vi "CSE - Execute Script (Basic).vi"(4 "Breakpoints":i32[](array[numeric]), 6 "exec parameters":T3={"pause counter"=1000, "pause, ms"=0, "autoVar"=TRUE, "enCpx"=TRUE}, 7 "VC Handle":T6=-1, 8 "error in":errorcluster, 9 "Run mode":T2 items=["Execute", "Abort", "Run", "Step", "Step Over", "Step Out", "Run (LM)", "Step (LM)", "Step Over (LM)", "Step Out (LM)", "unsupported"], 10 "Stm Index":i32, 11 "CSE RefNum":T4) -> (0 "error out":errorcluster, 1 "Stop Reason":T1=1 items=["Exec Start", "Action completed", "pause to breath", "reserved 1", "reserved 2", "custom"], 2 "Stm Index out":i32, 3 "dup CSE RefNum":T4, 5 "return value":dbl)   [LabVIEW 2021]
doc: "This VI is the basic CSE script executor. You can use it to run a parsed script, or you can create your own script engine based on it. Refer to the VI help for more details.\n\nIf <b>Run mode</b> is 0 (Execute), the VI completely executes a script starting from the <b>Stm Index</b> position (statement index) in regular mode with debugging disabled. Otherwise, the VI stops if either the specified action is completed or a breakpoint is reached.\n\n<b>Stm Index</b> specifies the initial index of the statement in a parsed script to execute.\n\n<b>Stm Index out</b> indicator returns the index of the statement to be performed next. When a script completes, <b>Stm Index out</b> returns -1.\n\n<b>Stop Reason</b> indicates the reason for the VI stop. The VI can return either 1 (Action completed) or 2 (pause to breath). All other values are reserved for compatibility with the \"Call Reason\" control of a Callback VI.\n\n<b>NOTE</b>: This VI never finishes until it completely executes a statement; it cannot return in the middle of a statement processing. This is true even if a statement involves calls to FuncVI functions.\n\n::: CalcExpress Toolkit :::\nCopyright (c) 2000-2026 Konstantin Shifershteyn. All rights reserved."
uses:
  cetypes.llb/VarMan Variable Context Handle.ctl
  cetypes.llb/CalcExpress Instance RefNum.ctl
  CSE Instance RefNum.ctl
  CSE Type - Run Mode.ctl
  CSE Type - Callback Call Reason.ctl
  cersrc/celveng32.dll
panel:
  in  "CE RefNum Tmpl":T5
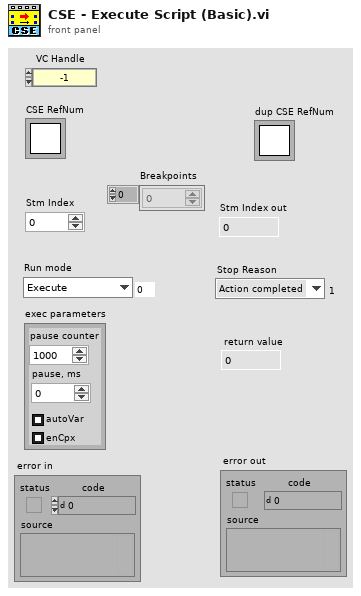
[diagram p1: front panel]
types:
  T1 = typedef "CSE Type - Callback Call Reason.ctl" = u32
  T2 = typedef "CSE Type - Run Mode.ctl" = u32
  T3 = cluster{"pause counter":i32, "pause, ms":i32, "autoVar":bool, "enCpx":bool}
  T4 = typedef "CSE Instance RefNum.ctl" = refnum<k1>
  T5 = typedef "CalcExpress Instance RefNum.ctl" = refnum<k1>
  T6 = typedef "VarMan Variable Context Handle.ctl" = i32
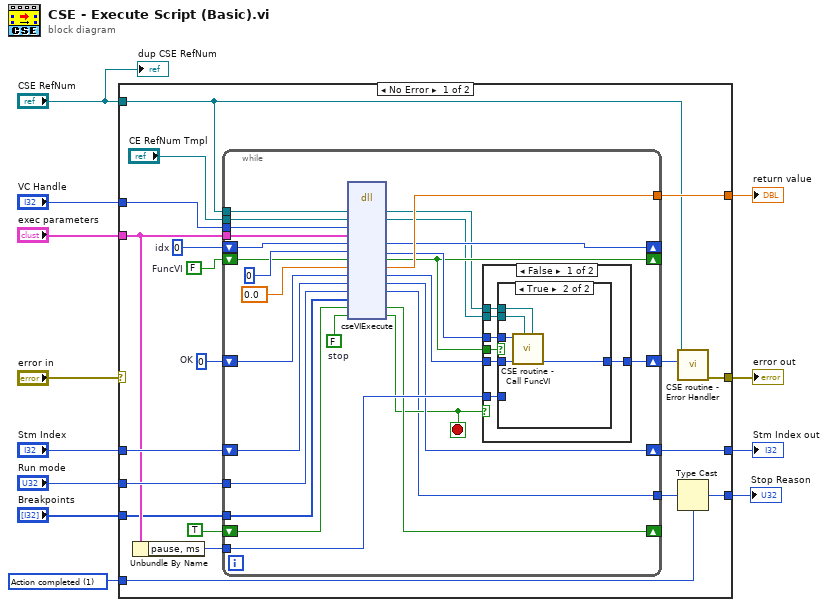
[diagram p0: block diagram]
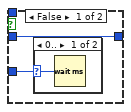
[diagram p2: hidden frame]
diagram:
  w1 = T1 1 items=["Exec Start", "Action completed", "pause to breath", "reserved 1", "reserved 2", "custom"] ("Stop Reason")
  n1 = case shown="No Error" "error in" {
    selector: "error in" -> [_ w77]
    tunnel: "VC Handle" -> [w30 _]
    tunnel: [w29 _] -> w11
    tunnel: [w28 w76] -> w10
    tunnel: "Stm Index" -> [w27 w76]
    tunnel: "CSE RefNum" -> [w20 _]
    tunnel: "Run mode" -> [w23 _]
    tunnel: "exec parameters" -> [w22 _]
    tunnel: [w19 w77] -> w5
    tunnel: "Breakpoints" -> [w16 _]
    tunnel: [w14 w75] -> w2
    tunnel: w1 -> [w13 w75]
    frame No Error {
      w24 = FALSE  # FuncVI
      w26 = 0  # OK
      w31 = 0  # idx
      n2 = Unbundle By Name(w22) -> ("pause, ms"=w25:i32)
      n3 = while {
        shift-left: w27 -> [w45]
        shift-right: [w43] -> w28
        tunnel: [w50] -> w29
        tunnel: w20 -> [w52]
        tunnel: w30 -> [w54]
        tunnel: "CE RefNum Tmpl" -> [w53]
        tunnel: w22 -> [w42]
        shift-left: w31 -> [w41]
        shift-right: [w40] -> _
        shift-left: w26 -> [w57]
        shift-right: [w58] -> w21
        tunnel: w25 -> [w48]
        shift-right: [w46] -> _
        shift-left: w24 -> [w47]
        tunnel: w23 -> [w44]
        shift-right: [w37] -> _
        shift-left: TRUE -> [w39]
        tunnel: w16 -> [w35]
        tunnel: [w34] -> w15
        stop <- w36 stop-if-true
        w38 = FALSE  # stop
        n4 = dll-call lib="C:/LV Projects/CalcExpress 40 LV2021/vi.lib/addons/CalcExpress/cersrc/celveng*.dll" fn="cseVIExecute" ("viCESPExecute")("iCESP"=w52, "iCE"=w53, "vch"=w54, "ExecPars"=w42, "expIdx"=w41, "expPNum"=0, "FuncVI"=w47, "retVal"=0.0 ("numeric value"), "ExecStat"=w57, "StmIdx"=w45, "Mode/Reason"=w44, "bpArray"=w35, "FirstTime"=w39, "stop"=w38) -> ("iCESP"=w32:T4, "iCE"=w33:T5, "expIdx"=w40:i32, "expPNum"=w49:i32, "FuncVI"=w46:bool, "retVal"=w50:dbl, "ExecStat"=w51:i32, "StmIdx"=w43:i32, "Mode/Reason"=w34:T2, "FirstTime"=w37:bool, "stop"=w36:bool)  [unwired: 7 in, 2 out]
        n5 = case shown="False" w36 {
          tunnel: [w65 w74] -> w58
          tunnel: w51 -> [w64 w74]
          tunnel: w49 -> [w63 _]
          tunnel: w46 -> [w62 _]
          tunnel: w48 -> [w61 _]
          tunnel: w33 -> [w60 _]
          tunnel: w32 -> [w59 _]
          frame False {
            n6 = case shown="True" w62 {
              tunnel: [w67 w71] -> w65
              tunnel: w64 -> [w67 w72]
              tunnel: w63 -> [_ w73]
              tunnel: w61 -> [w66 _]
              tunnel: w60 -> [_ w70]
              tunnel: w59 -> [_ w69]
              frame False {
                n7 = case shown="0.." w66 {
                  selector: w66 -> [w68 _]
                  frame 0.. {
                    n8 = Wait (ms)(milliseconds to wait=w68) -> ()  [unwired: 1 out]
                  }
                  frame ..-1 {
                  }
                }
              }
              frame True {
                n9 = call "CSE routine - Call FuncVI.vi"("CSE RefNum"=w69, "CE InstanceRef"=w70, "error code"=w72, "ParNum"=w73) -> ("error code out"=w71:i32)  [unwired: 5 in]
              }
            }
          }
          frame True {
          }
        }
      }
      n10 = call "CSE routine - Error Handler.vi"("exec status"=w21, "CSE RefNum"=w20) -> ("error out"=w19:errorcluster)  [unwired: 5 in, 2 out]
      n11 = Type Cast(type=w13, x=w15) -> (*(type *) &x=w14:T1)
    }
    frame Error {
    }
  }
  "return value" <- w11
  "Stm Index out" <- w10
  "error out" <- w5
  "Stop Reason" <- w2
  "dup CSE RefNum" <- "CSE RefNum"
